vi "libssh2_knownhost_get.vi"(8 "error in (no error)":errorcluster, 10 "previous host key":T1, 11 "host key database":T2) -> (0 "error out":errorcluster, 1 "end reached":bool, 2 "host key":T1)   [LabVIEW 2017, in "libssh2.lvlib"]
doc: "Get a host key from a host key database. Returns the first host key from the database when <B>previous</B> is unwired.\n\n<B>end reached</B> is TRUE when the final host key is reached. Otherwise, FALSE."
uses:
  libssh2.lvlib
  Host Key Database Refnum.ctl
  Host Key Refnum.ctl
  Not A Host Key Database.vi
  <vilib>/Utility/error.llb/Error Cluster From Error Code.vi
  Global Settings.vi
  Read Host Key Database Refnum.vi
  <vilib>/Utility/semaphor.llb/Acquire Semaphore.vi
  <vilib>/Utility/semaphor.llb/Release Semaphore.vi
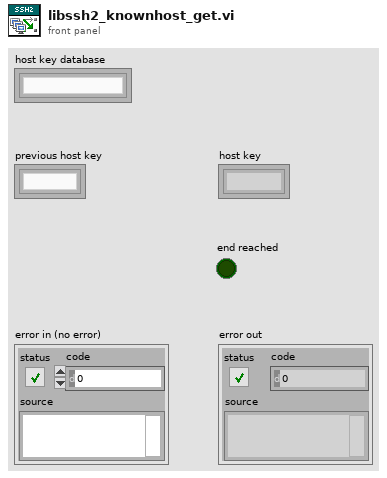
[diagram p1: front panel]
types:
  T1 = typedef "libssh2.lvlib/Host Key Refnum.ctl" = refnum<k1>
  T2 = typedef "libssh2.lvlib/Host Key Database Refnum.ctl" = refnum<k1>
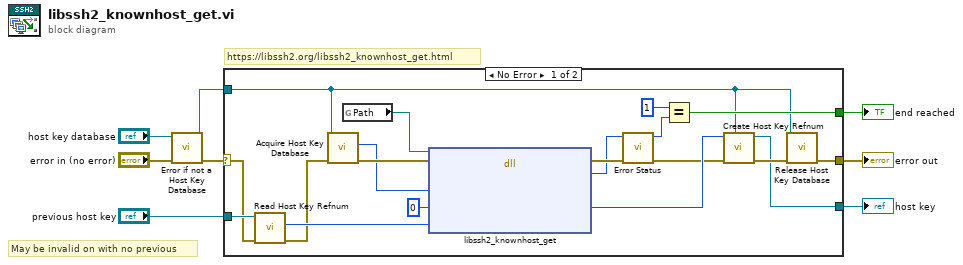
[diagram p0: block diagram]
diagram:
  # "May be invalid on with no previous"
  # "https://libssh2.org/libssh2_knownhost_get.html"
  n1 = call "Error if not a Host Key Database.vi"("error in (no error)"="error in (no error)", "host key database"="host key database") -> ("error out"=w4:errorcluster, "host key database out"=w2:T2)  [unwired: 8 in]
  n2 = case shown="No Error" w4 {
    selector: w4 -> [w24 w28]
    tunnel: [w10 w28] -> w8
    tunnel: w2 -> [w9 _]
    tunnel: "previous host key" -> [w26 _]
    tunnel: [w25 _] -> w7
    tunnel: [w23 _] -> w5
    frame No Error {
      n3 = call "Read Host Key Refnum.vi"("error in (no error)"=w24, "host key"=w26) -> ("error out"=w17:errorcluster, "libssh2_knownhost*"=w19:u64)  [unwired: 7 in, 1 out]
      n4 = call "Acquire Host Key Database.vi"("error in (no error)"=w17, "host key database"=w9) -> ("error out"=w21:errorcluster, "LIBSSH2_KNOWNHOSTS*"=w20:u64)  [unwired: 8 in]
      n5 = global read "Global Settings.vi" "Path"() -> (w16:path)
      n6 = dll-call lib="?" fn="libssh2_knownhost_get"(path in=w16, error in=w21, "hosts"=w20, "store"=u64 0, "prev"=w19) -> (error out=w22:errorcluster, "return value"=w14:i32, "store"=w18:u64)  [unwired: 3 in, 1 out]
      n7 = call "Error Status.vi"("error in (no error)"=w22, "return value"=w14) -> ("error out"=w15:errorcluster, "return value out"=w12:i32)  [unwired: 8 in]
      n8 = Equal?(x=1, y=w12) -> (x = y?=w23:bool)
      n9 = call "Create Host Key Refnum.vi"("host key database"=w9, "error in (no error)"=w15, "libssh2_knownhost*"=w18) -> ("error out"=w27:errorcluster, "host key"=w25:T1)  [unwired: 7 in]
      n10 = call "Release Host Key Database.vi"("error in (no error)"=w27, "host key database"=w9) -> ("error out"=w10:errorcluster)  [unwired: 9 in]
    }
    frame Error {
    }
  }
  "error out" <- w8
  "host key" <- w7
  "end reached" <- w5
